vi "GetDC Wrapper Template.vi"(0 "hWnd":u64, 11 "error in":errorcluster) -> (4 "HDC":u64, 15 "error out":errorcluster)   [LabVIEW 2020]
doc: "Returns a device context for the client area of hWnd, or for the whole screen when hWnd is 0, through user32.dll GetDC (stdcall, called in any thread). Every HDC obtained here must be given back with user32 ReleaseDC.vi. When error in carries an error the DLL is not called. Generated by scripts\\Build Win32 Wrappers.vi - do not edit by hand, rebuild it."
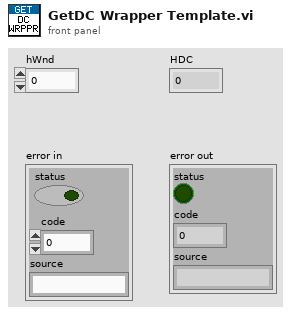
[diagram p1: front panel]
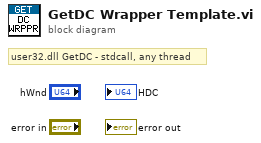
[diagram p0: block diagram]
diagram:
  # "user32.dll GetDC - stdcall, any thread"
